vi "Write Decel_ms_krpm.vi"(8 "error in (no error)":errorcluster, 10 "Decel_ms_krpm":i32, 11 "ServoDrive in":refnum<class "ServoDrive.lvclass">) -> (0 "error out":errorcluster, 3 "ServoDrive out":refnum<class "ServoDrive.lvclass">)   [LabVIEW 2021, in "ServoDrive.lvclass"]
uses:
  ServoDrive.lvclass
  ServoDrive.lvclass/ServoDrive.ctl
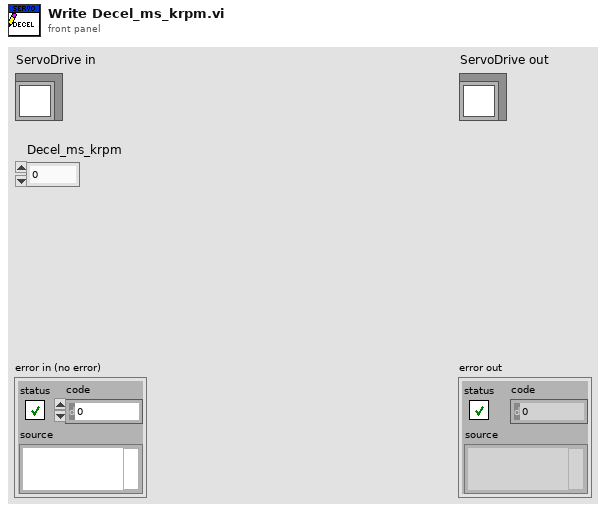
[diagram p1: front panel]
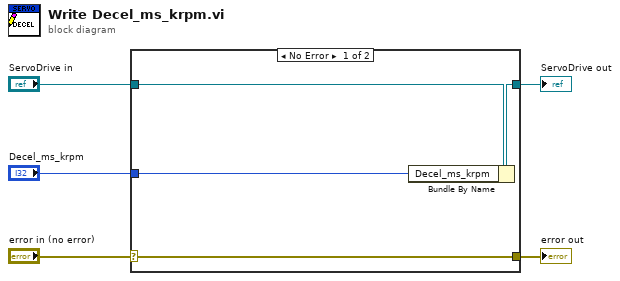
[diagram p0: block diagram]
diagram:
  n1 = case shown="No Error" "error in (no error)" {
    selector: "error in (no error)" -> [w9 w10]
    tunnel: [w9 w10] -> w4
    tunnel: [w7 w11] -> w2
    tunnel: "ServoDrive in" -> [w8 w11]
    tunnel: "Decel_ms_krpm" -> [w6 _]
    frame No Error {
      n2 = Bundle By Name(cluster=w8, "Decel_ms_krpm"=w6) -> (w7:refnum<class "ServoDrive.lvclass">)
    }
    frame Error {
    }
  }
  "error out" <- w4
  "ServoDrive out" <- w2
